vi "VHist - Extrapolate history values.vi"(4 "points":i32=1, 6 "method (linear)":T1(ring), 8 "error in":errorcluster, 9 "time (0: now)":dbl format="%<%H:%M:%S%2u\n%d/%m/%Y>T", 10 "history data":dbl[](array[numeric]) format="%.2f", 11 "time stamps":dbl[](array[numeric]) format="%<%H:%M:%S%2u\n%d/%m/%Y>T") -> (0 "error out":errorcluster, 2 "history data out":dbl[](array[numeric]) format="%.2f", 3 "time stamps out":dbl[](array[numeric]) format="%<%H:%M:%S%2u\n%d/%m/%Y>T")   [LabVIEW 2021]
doc: "::: CalcExpress Toolkit :::\nCopyright (c) 2000-2026 Konstantin Shifershteyn. All rights reserved."
uses:
  <vilib>/Analysis/NI_AALPro.lvlib
panel:
  # "The VI requires the historiy to be arranged\nin increasing timestamp order."
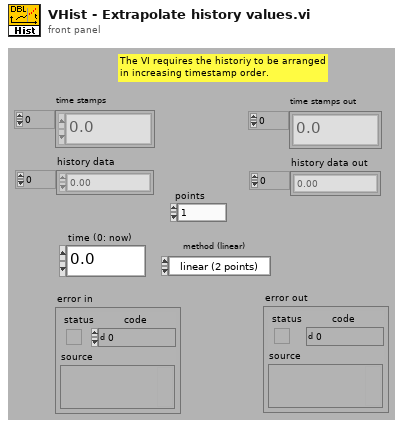
[diagram p1: front panel]
types:
  T1 = enum16{"linear (2 points)", "polynominal", "rational", "spline"}
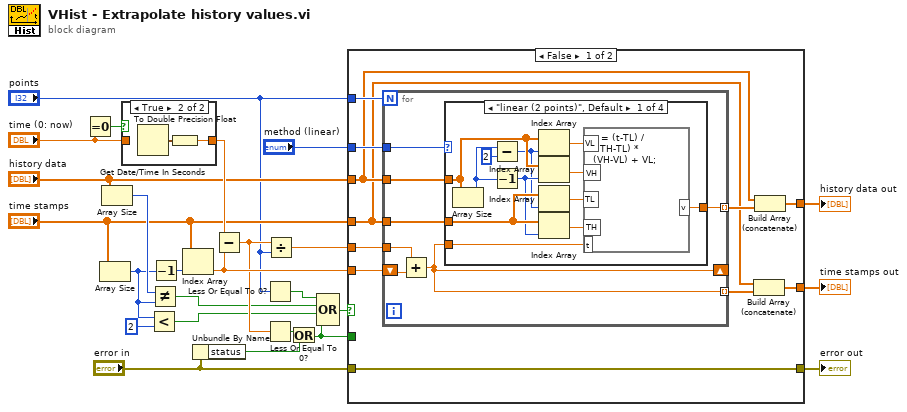
[diagram p0: block diagram]
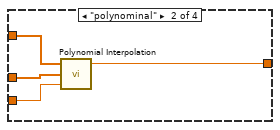
[diagram p2: hidden frame]
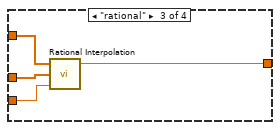
[diagram p3: hidden frame]
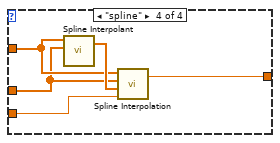
[diagram p4: hidden frame]
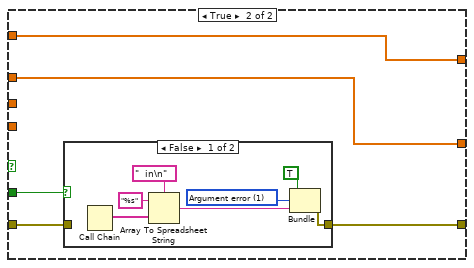
[diagram p5: hidden frame]
diagram:
  n1 = Equal To 0?(x="time (0: now)") -> (x = 0?=w25:bool)
  n2 = Array Size(array="time stamps") -> (size(s)=w12:i32)
  n3 = Array Size(array="history data") -> (size(s)=w13:i32)
  n4 = case shown="True" w25 {
    tunnel: [w26 w28] -> w22
    tunnel: "time (0: now)" -> [w26 _]
    frame False {
    }
    frame True {
      n5 = Get Date/Time In Seconds() -> (seconds since 1Jan1904=w27:timestamp)
      n6 = To Double Precision Float(number=w27) -> (double precision float=w28:dbl)
    }
  }
  n7 = Less?(x=w12, y=2) -> (x < y?=w9:bool)
  n8 = Not Equal?(x=w13, y=w12) -> (x != y?=w10:bool)
  n9 = Decrement(x=w12) -> (x-1=w23:i32)
  n10 = Index Array(array="time stamps", index=w23) -> (element=w21:dbl)
  n11 = Unbundle By Name("error in") -> ("status"=w15:bool)
  n12 = Subtract(x=w22, y=w21) -> (x-y=w19:dbl)
  n13 = Less Or Equal To 0?(x="points") -> (x <= 0?=w16:bool)
  n14 = Less Or Equal To 0?(x=w19) -> (x <= 0?=w17:bool)
  n15 = Divide(x=w19, y="points") -> (x/y=w20:dbl)
  n16 = Or(x=w17, y=w15) -> (x .or. y?=w14:bool)
  n17 = Compound Arithmetic op=OR(w16, w10, w9, w14) -> (w8:bool)
  n18 = case shown="False" w8 {
    tunnel: w21 -> [w39 _]
    tunnel: w20 -> [w38 _]
    tunnel: "points" -> [w37 _]
    tunnel: "method (linear)" -> [w36 _]
    tunnel: "time stamps" -> [w32 w75]
    tunnel: "history data" -> [w33 w76]
    tunnel: [w31 w76] -> w2
    tunnel: [w30 w75] -> w3
    tunnel: w14 -> [_ w73]
    tunnel: [w29 w72] -> w6
    tunnel: "error in" -> [w29 w74]
    frame False {
      n19 = for {
        N: w37 -> [_]
        shift-right: [w40] -> _
        shift-left: w39 -> [w46]
        tunnel: w38 -> [w45]
        tunnel: w36 -> [w44]
        tunnel: w32 -> [w43]
        tunnel: w33 -> [w42]
        tunnel: [w41] -> w35 mode=indexing
        tunnel: [w40] -> w34 mode=indexing
        n20 = Add(x=w45, y=w46) -> (x+y=w40:dbl)
        n21 = case shown="\"linear (2 points)\", Default" w44 {
          tunnel: w43 -> [w56 w62 w65 w68]
          tunnel: w40 -> [w58 w61 w64 w70]
          tunnel: w42 -> [w55 w60 w66 w69]
          tunnel: [w57 w59 w63 w67] -> w41
          frame "linear (2 points)", Default {
            n22 = Array Size(array=w55) -> (size(s)=w54:i32)
            n23 = Subtract(x=w54, y=2) -> (x-y=w51:i32)
            n24 = Decrement(x=w54) -> (x-1=w52:i32)
            n25 = Index Array(array=w55, index=w51) -> (element=w50:dbl)
            n26 = Index Array(array=w55, index=w52) -> (element=w49:dbl)
            n27 = Index Array(array=w56, index=w51) -> (element=w48:dbl)
            n28 = Index Array(array=w56, index=w52) -> (element=w47:dbl)
            n29 = formula code="v = (t-TL) /\n (TH-TL) * \n(VH-VL) + VL;"("TH"=w47, "TL"=w48, "VH"=w49, "VL"=w50, "t"=w58) -> ("v"=w57:dbl)
          }
          frame "polynominal" {
            n30 = call <vilib>:"Polynomial Interpolation.vi"("x value"=w61, "X"=w62, "Y"=w60) -> ("interpolation value"=w59:dbl)  [unwired: 2 out]
          }
          frame "rational" {
            n31 = call <vilib>:"Rational Interpolation.vi"("x value"=w64, "X"=w65, "Y"=w66) -> ("interpolation value"=w63:dbl)  [unwired: 2 out]
          }
          frame "spline" {
            n32 = call <vilib>:"Spline Interpolant.vi"("X"=w68, "Y"=w69) -> ("Interpolant"=w71:dbl[])  [unwired: 2 in, 1 out]
            n33 = call <vilib>:"Spline Interpolation.vi"("x value"=w70, "Interpolant"=w71, "X"=w68, "Y"=w69) -> ("interpolation value"=w67:dbl)  [unwired: 1 out]
          }
        }
      }
      n34 = Build Array (concatenate)(w32, w34) -> (w30:dbl[])
      n35 = Build Array (concatenate)(w33, w35) -> (w31:dbl[])
    }
    frame True {
      n36 = case shown="False" w73 {
        tunnel: [w83 w84] -> w72
        tunnel: w74 -> [_ w84]
        frame False {
          w81 = 1 items=["No error", "Argument error", "Memory is full", "Out of zone", "End of file", "File already open", "Generic file I/O error", "File not found", "File permission error", "Disk is full", "Duplicate path", "Too many files open", "System feature not enabled", "Resource file not found", "Cannot add resource", "Resource not found", "Image not found", "Image memory error", "Pen does not exist", "Config type invalid", "Config token not found", "Config parse error", "Config memory error", "Bad external code format", "Bad external code offset", "External code not present", "Null window", "Destroy window error", "Null menu", "Print aborted", "Bad print record", "Print driver error", "Windows error during printing", "Memory error during printing", "Print dialog error", "Generic print error", "Invalid device refnum", "Device not found", "Device parameter error", "Device unit error", "Cannot open device", "Device call aborted", "Generic error", "Cancelled by user", "Object ID too low", "Object ID too high", "Object not in heap", "Unknown heap", "Unknown object (invalid DefProc)", "Unknown object (DefProc not in table)", "Message out of range", "Invalid (null) method", "Unknown message", "Manager call not supported", "Bad address", "Network operation in progress", "Network operation timed out", "Connection is busy", "Network attribute not supported", "Network error", "Address in use", "System out of memory", "Connection aborted", "Connection refused", "Not connected", "Already connected", "Connection closed", "Initialization error (interapplication manager)", "Bad occurrence", "Wait on unbound occurrence handler", "Occurrence queue overflow", "Datalog type conflict", "Unused", "Unrecognized type (interapplication manager)", "Memory corrupt", "Failed to make temporary DLL", "Old CIN version", "Drag socket not found", "Failed to load drop-object", "Failed to register OLE object", "Failed to release OLE object", "Format specifier type mismatch", "Unknown format specifier", "Too few format specifiers", "Too many format specifiers", "Scan failed", "Newer CIN version", "Error converting to variant", "Runtime menu error", "Password tampered", "Variant attribute not found", "Incompatible variant data type", "Event data is not available", "Event Store is not present", "Occurrence is not found", "Event Queue is not created", "Event info is not available", "Refnum passed is NULL", "Error retrieving Class GUID", "Error retrieving CoClass GUID", "Error retrieving TypeLib GUID.", "Bad built application magic bytes.", "Specific driver is different from the specific driver associated with the Logical Name.", "There is no session opened to the class driver.", "Max Error", "MAX - Error with config objects", "MAX - Error loading configuration", "MAX - Group not supported"]
          n37 = Call Chain() -> (call chain=w80:string[])
          n38 = Array To Spreadsheet String(delimiter (Tab)="  in\n", array=w80, 3:"%s" ("format string")) -> (spreadsheet string=w77:string)
          n39 = Bundle(TRUE, w81, "spreadsheet string"=w77) -> (w83:cluster{bool, i32, "spreadsheet string":string})  [unwired: 1 in]
        }
        frame True {
        }
      }
    }
  }
  "error out" <- w6
  "time stamps out" <- w3
  "history data out" <- w2
